vi "QuickDrop Plugin.vi"(6 "Variant in":variant, 7 "Shift Pressed?":bool, 8 "error in (no error)":errorcluster, 10 "QD Combo Box Ref":refnum<vi>, 11 "QD Launch VI Ref":refnum<vi>) -> (0 "error out":errorcluster, 4 "Variant out":variant)   [LabVIEW 2020]
doc: "Run all LUnit tests in memory which call the current VI. Hold Shift to run all tests in current project.\n\nDefault Shortcut - [L]"
uses:
  0b8230da-52ab-4c04-9608-fd4c63fdf1a3.vi
  LUnit Test Case.lvclass
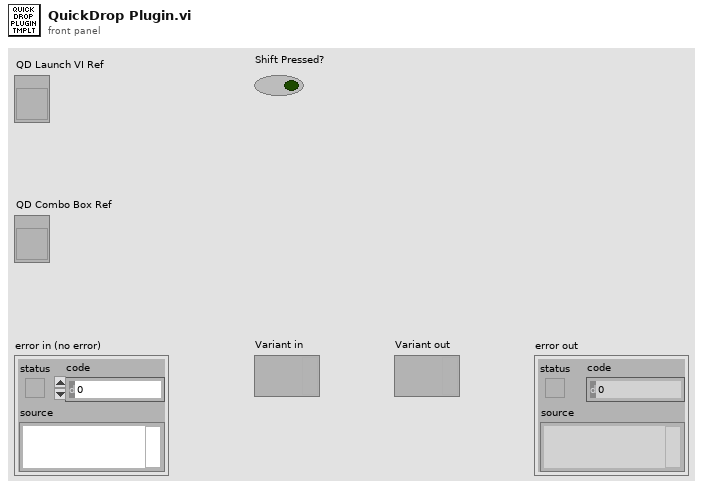
[diagram p1: front panel]
types:
  T1 = enum32{"Invalid", "Standard", "Closed", "Hidden", "Minimized", "Maximized"}
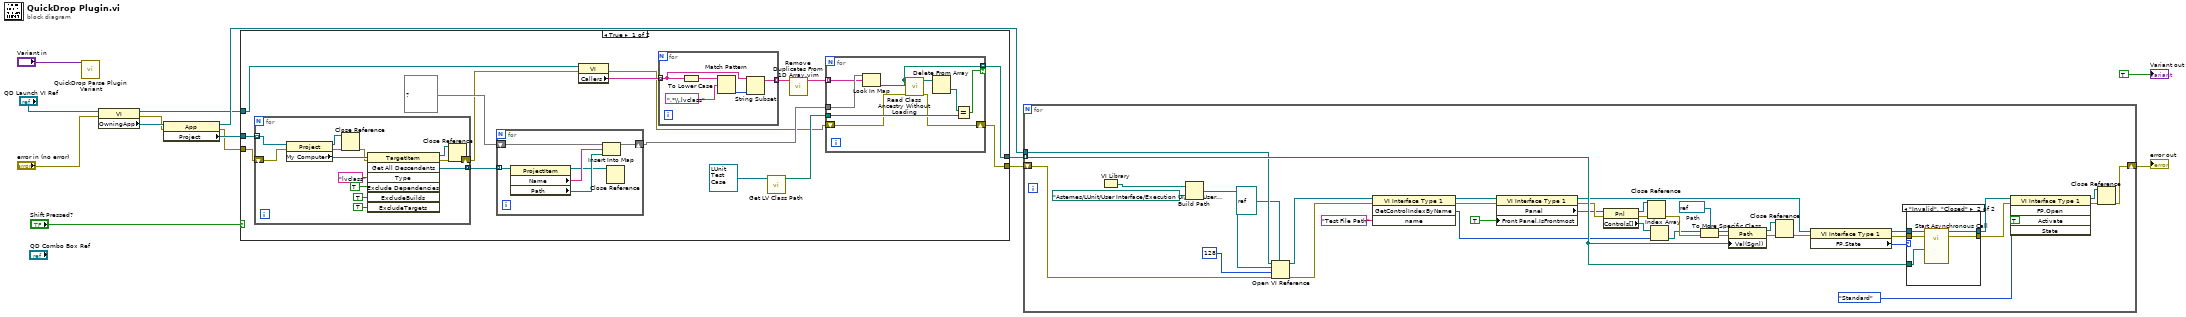
[diagram p0: block diagram]
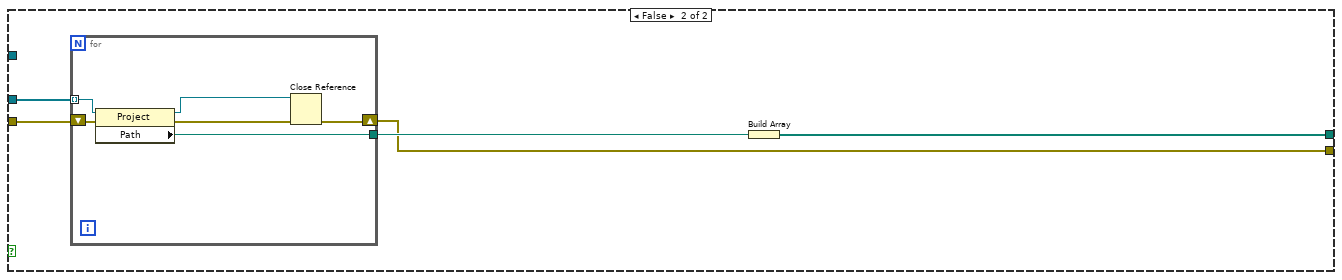
[diagram p2: hidden frame]
diagram:
  n1 = call <vilib>:"QuickDrop Parse Plugin Variant.vi"("QDKS Variant in"="Variant in") -> ()  [unwired: 12 in, 3 out]
  n2 = property class="VI"(reference="QD Launch VI Ref", error in="error in (no error)") -> (reference out=w1:refnum<vi>, error out=w6:errorcluster, "OwningApp"=w10:refnum<vi>)
  n3 = property class="App"(reference=w10, error in=w6) -> (reference out=w2:refnum<vi>, error out=w7:errorcluster, "Project"=w8:refnum<vi>[])
  n4 = case shown="True" "Shift Pressed?" {
    tunnel: w8 -> [w21 w67]
    tunnel: w7 -> [w23 w66]
    tunnel: [w22 w65] -> w5
    tunnel: [w20 w64] -> w3
    tunnel: w1 -> [w19 _]
    frame True {
      n5 = for {
        tunnel: [w38] -> w29 mode=concatenating
        tunnel: w21 -> [w33] mode=indexing
        shift-right: [w31] -> w17
        shift-left: w23 -> [w36]
        n6 = property class="Project"(reference=w33, error in=w36) -> (reference out=w30:refnum<vi>, error out=w37:errorcluster, "My Computer"=w43:refnum<vi>)
        n7 = Close Reference(reference=w30, error in (no error)=w37) -> (error out=w35:errorcluster)
        n8 = invoke class="TargetItem" method="Get All Descendents"(reference=w43, error in=w35, "Type"="lvclass", "Exclude Dependencies"=TRUE ("ExcludeDependencies"), "ExcludeBuilds"=TRUE, "ExcludeTargets"=TRUE) -> (reference out=w34:refnum<vi>, error out=w32:errorcluster, "All Descendents"=w38:refnum<vi>[])  [unwired: 1 in, 4 out]
        n9 = Close Reference(reference=w34, error in (no error)=w32) -> (error out=w31:errorcluster)
      }
      n10 = for {
        tunnel: w29 -> [w49] mode=indexing
        shift-right: [w45] -> w24
        shift-left: map{string, path} {} ("map") -> [w46]
        n11 = property class="ProjectItem"(reference=w49) -> (reference out=w44:refnum<vi>, "Name"=w48:string, "Path"=w47:path)  [unwired: 1 in, 1 out]
        n12 = Insert Into Map(map in=w46, key=w48, value=w47) -> (map out=w45:map{string, path})  [unwired: 2 out]
        n13 = Close Reference(reference=w44) -> ()  [unwired: 1 in, 1 out]
      }
      n14 = property class="VI"(reference=w19, error in=w17) -> (error out=w16:errorcluster, "Callers"=w18:string[])  [unwired: 1 out]
      n15 = for {
        tunnel: w18 -> [w61] mode=indexing
        tunnel: [w60] -> w27 mode=indexing
        n16 = To Lower Case(string=w61) -> (all lower case string=w63:string)
        n17 = Match Pattern(string=w63, regular expression=".*\\.lvclass") -> (offset past match=w62:i32)  [unwired: 1 in, 3 out]
        n18 = String Subset(string=w61, length (rest)=w62) -> (substring=w60:string)  [unwired: 1 in]
      }
      n19 = call <vilib>:"Get LV Class Path.vi"("object"=refnum<class "LUnit Test Case.lvclass"> refnum ("LUnit Test Case.lvclass")) -> ("class path"=w25:path)  [unwired: 9 in, 1 out]
      n20 = call "Remove Duplicates From 1D Array.vim"("array"=w27) -> ("array with duplicates removed"=w26:string[])  [unwired: 10 in]
      n21 = for {
        tunnel: w26 -> [w53] mode=indexing
        tunnel: w25 -> [w56]
        tunnel: [w52] -> w22 mode=indexing if=w55
        tunnel: w24 -> [w54]
        shift-right: [w51] -> w20
        shift-left: w16 -> [w50]
        n22 = Look In Map(map=w54, key=w53) -> (value=w52:path)  [unwired: 1 in, 1 out]
        n23 = call <vilib>:"Read Class Ancestry Without Loading.vi"("error in (no error)"=w50, "LabVIEW Class Path"=w52) -> ("error out"=w51:errorcluster, "Class Ancestry"=w58:path[])  [unwired: 8 in]
        n24 = Delete From Array(array=w58) -> (deleted portion=w57:path)  [unwired: 2 in, 1 out]
        n25 = Equal?(x=w57, y=w56) -> (x = y?=w55:bool)
      }
    }
    frame False {
      n26 = for {
        tunnel: [w74] -> w68
        tunnel: w67 -> [w70] mode=indexing
        shift-right: [w69] -> w64
        shift-left: w66 -> [w72]
        n27 = property class="Project"(reference=w70, error in=w72) -> (reference out=w71:refnum<vi>, error out=w73:errorcluster, "Path"=w74:path)
        n28 = Close Reference(reference=w71, error in (no error)=w73) -> (error out=w69:errorcluster)
      }
      n29 = Build Array(w68) -> (w65:path[])
    }
  }
  n30 = for {
    tunnel: w5 -> [w113] mode=indexing
    tunnel: w2 -> [w112]
    shift-right: [w111] -> w4
    shift-left: w3 -> [w110]
    w89 = refnum<vi> refnum  # Path
    n31 = VI Library() -> (path=w83:path)
    n32 = Build Path(base path=w83, name or relative path=path "Astemes/LUnit/User Interface/Execution UI/LUnit User Interface.vi" ("Relative Path from 1 to 2")) -> (appended path=w78:path)
    n33 = Open VI Reference(type specifier VI Refnum (for type only)=refnum<vi> refnum, application reference (local)=w112, vi path=w78, options=128, error in (no error)=w110) -> (vi reference=w101:refnum<vi>, error out=w102:errorcluster)  [unwired: 1 in]
    n34 = invoke class="VI Interface Type 1" method="GetControlIndexByName"(reference=w101, error in=w102, "name"="Test File Path" ("Control Name")) -> (reference out=w85:refnum<vi>, error out=w95:errorcluster, "GetControlIndexByName"=w88:i32)  [unwired: 1 in, 1 out]
    n35 = property class="VI Interface Type 1"(reference=w85, error in=w95, "Front Panel.IsFrontmost"=TRUE ("Front Panel Window:Is Frontmost")) -> (reference out=w108:refnum<vi>, error out=w94:errorcluster, "Panel"=w84:refnum<vi>)
    n36 = property class="Pnl"(reference=w84, error in=w94) -> (reference out=w98:refnum<vi>, error out=w93:errorcluster, "Controls[]"=w87:refnum<vi>[])
    n37 = Close Reference(reference=w98, error in (no error)=w93) -> (error out=w97:errorcluster)
    n38 = Index Array(array=w87, index=w88) -> (element=w91:refnum<vi>)
    n39 = To More Specific Class(target class=w89, reference=w91, error in=w97) -> (specific class reference=w90:refnum<vi>, error out=w92:errorcluster)
    n40 = property class="Path"(reference=w90, error in=w92, "Val(Sgnl)"=w113) -> (reference out=w99:refnum<vi>, error out=w96:errorcluster)
    n41 = Close Reference(reference=w99, error in (no error)=w96) -> (error out=w106:errorcluster)
    n42 = property class="VI Interface Type 1"(reference=w108, error in=w106) -> (reference out=w104:refnum<vi>, error out=w103:errorcluster, "FP.State"=w105:T1)
    n43 = case shown="\"Invalid\", \"Closed\"" w105 {
      tunnel: w103 -> [w115 w120]
      tunnel: w104 -> [w114 w119]
      tunnel: [w115 w117] -> w107
      tunnel: [w114 w118] -> w109
      tunnel: w113 -> [_ w116]
      frame Default {
      }
      frame "Invalid", "Closed" {
        n44 = call-by-ref "Start Asynchronous Call"(reference=w119, error in=w120, "Test File Path"=w116) -> (reference out=w118:refnum<vi>, error out=w117:errorcluster)  [unwired: 11 in]
      }
    }
    n45 = invoke class="VI Interface Type 1" method="FP.Open"(reference=w109, error in=w107, "Activate"=TRUE ("Activate?"), "State"=T1."Standard") -> (reference out=w79:refnum<vi>, error out=w80:errorcluster)  [unwired: 1 in, 3 out]
    n46 = Close Reference(reference=w79, error in (no error)=w80) -> (error out=w111:errorcluster)
  }
  "error out" <- w4
  "Variant out" <- TRUE
